vi "query Starting and Num RB.vi"(8 "error in (no error)":errorcluster, 10 "RB Setting Param":T1, 11 "LTE in":refnum<class "LTE.lvclass">) -> (0 "error out":errorcluster, 2 "RB Value":i32, 3 "LTE out":refnum<class "LTE.lvclass">)   [LabVIEW 2023, in "ANRITSU Call Box.lvlib" / "LTE.lvclass"]
uses:
  LTE.lvclass
  LTE.lvclass/LTE.ctl
  ANRITSU Call Box.lvlib
  Type Definition/LTE RB Setting Params for query.ctl
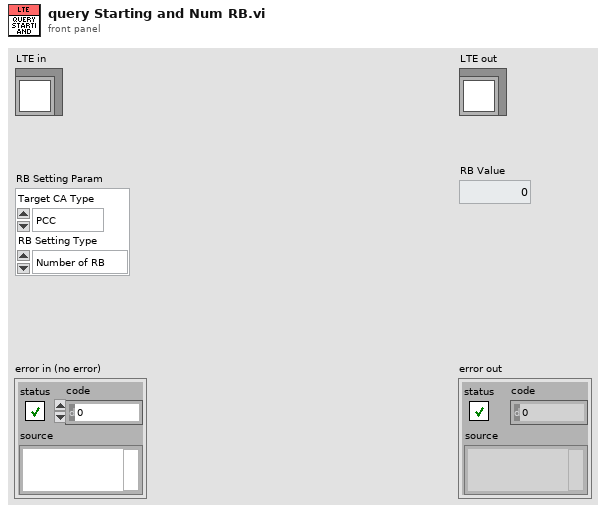
[diagram p1: front panel]
types:
  T1 = typedef "ANRITSU Call Box.lvlib/LTE RB Setting Params for query.ctl" = cluster{"Target CA Type":enum16{"PCC", "SCC1"}, "RB Setting Type":enum16{"Number of RB", "Starting RB"}}
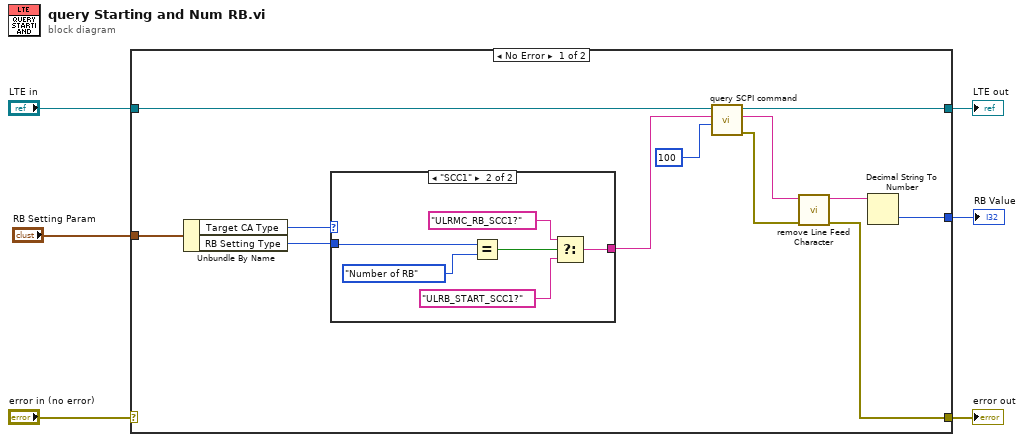
[diagram p0: block diagram]
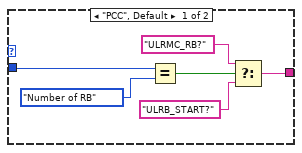
[diagram p2: hidden frame]
diagram:
  n1 = case shown="No Error" "error in (no error)" {
    selector: "error in (no error)" -> [_ w32]
    tunnel: [w7 w32] -> w5
    tunnel: [w12 w31] -> w3
    tunnel: "LTE in" -> [w15 w31]
    tunnel: "RB Setting Param" -> [w16 _]
    tunnel: [w8 _] -> w1
    frame No Error {
      n2 = Unbundle By Name(w16) -> ("Target CA Type"=w18:enum16{"PCC", "SCC1"}, "RB Setting Type"=w17:enum16{"Number of RB", "Starting RB"})
      n3 = case shown="\"SCC1\"" w18 {
        tunnel: w17 -> [w24 w30]
        tunnel: [w19 w25] -> w14
        frame "PCC", Default {
          n4 = Equal?(x=w24, y=enum16{"Number of RB", "Starting RB"}."Number of RB") -> (x = y?=w22:bool)
          n5 = Select(t="ULRMC_RB?" ("string"), s=w22, f="ULRB_START?" ("string")) -> (s? t:f=w19:string)
        }
        frame "SCC1" {
          n6 = Equal?(x=w30, y=enum16{"Number of RB", "Starting RB"}."Number of RB") -> (x = y?=w28:bool)
          n7 = Select(t="ULRMC_RB_SCC1?" ("string"), s=w28, f="ULRB_START_SCC1?" ("string")) -> (s? t:f=w25:string)
        }
      }
      n8 = call "query SCPI command.vi"("Read Buffer Length"=u32 100, "SCPI Command"=w14, "LTE in"=w15) -> ("error out"=w11:errorcluster, "Read Buffer String"=w10:string, "LTE out"=w12:refnum<class "LTE.lvclass">)  [unwired: 6 in]
      n9 = call "remove Line Feed Character.vi"("error in"=w11, "Query String"=w10) -> ("error out"=w7:errorcluster, "Line Feed Removed String"=w9:string)  [unwired: 8 in]
      n10 = Decimal String To Number(string=w9) -> (number=w8:i32)  [unwired: 2 in, 1 out]
    }
    frame Error {
    }
  }
  "error out" <- w5
  "LTE out" <- w3
  "RB Value" <- w1
